vi "Replace String in File.vi"(7 "File Path":path, 8 "error in":errorcluster, 9 "Replace String":string, 10 "Search String":string, 11 "IFile Manager in":refnum<class "Mock IFile Manager.lvclass">) -> (0 "error out":errorcluster, 3 "IFile Manager out":refnum<class "Mock IFile Manager.lvclass">)   [LabVIEW 2026, in "Mock IFile Manager.lvclass"]
doc: "This VI replaces all instances of the search string by the replace strin in the provided text file."
uses:
  Mock IFile Manager.lvclass
  C:/Program Files/National Instruments/LabVIEW 2026/vi.lib/Astemes/LMock/Mock.lvclass
  Mock IFile Manager.lvclass/Mock IFile Manager.ctl
  <vilib>/Astemes/LMock/Mock.lvclass
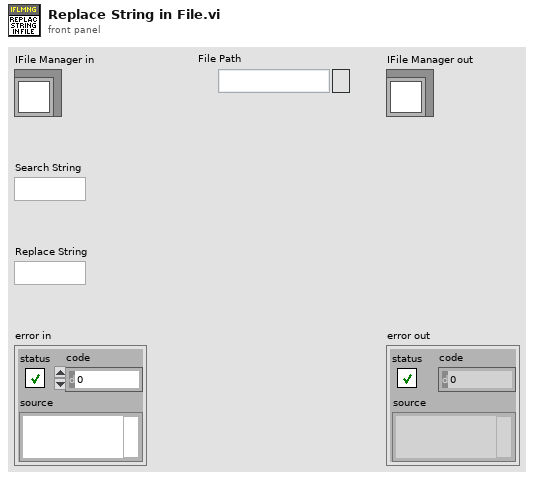
[diagram p1: front panel]
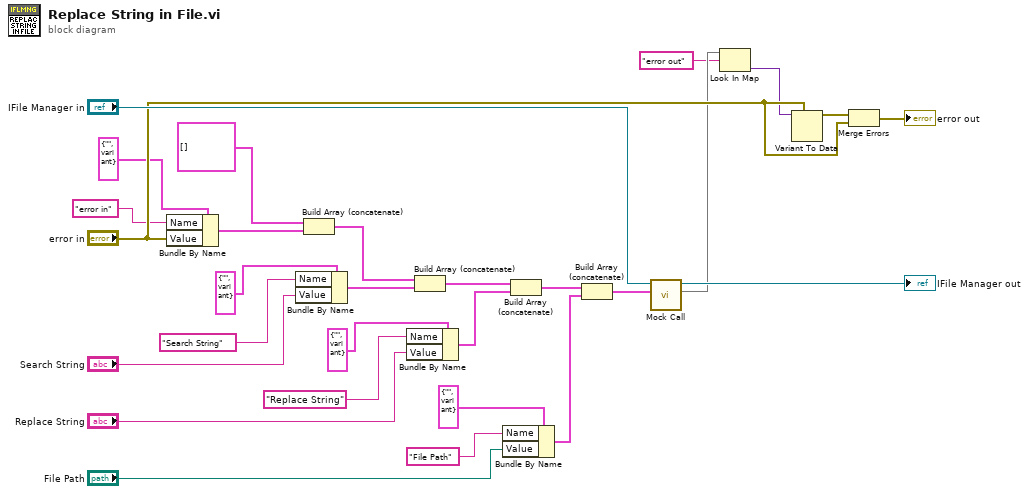
[diagram p0: block diagram]
diagram:
  n1 = Bundle By Name(cluster=cluster{"Name":string, "Value":variant} {"Name"="", "Value"=variant} ("element"), "Name"="error in", "Value"="error in") -> (w7:cluster{"Name":string, "Value":variant})
  n2 = Bundle By Name(cluster=cluster{"Name":string, "Value":variant} {"Name"="", "Value"=variant} ("element"), "Name"="Search String", "Value"="Search String") -> (w5:cluster{"Name":string, "Value":variant})
  n3 = Build Array (concatenate)(cluster{"Name":string, "Value":variant}[] [] ("Control Values"), w7) -> (w16:cluster{"Name":string, "Value":variant}[])
  n4 = Bundle By Name(cluster=cluster{"Name":string, "Value":variant} {"Name"="", "Value"=variant} ("element"), "Name"="Replace String", "Value"="Replace String") -> (w3:cluster{"Name":string, "Value":variant})
  n5 = Build Array (concatenate)(w16, w5) -> (w19:cluster{"Name":string, "Value":variant}[])
  n6 = Bundle By Name(cluster=cluster{"Name":string, "Value":variant} {"Name"="", "Value"=variant} ("element"), "Name"="File Path", "Value"="File Path") -> (w1:cluster{"Name":string, "Value":variant})
  n7 = Build Array (concatenate)(w19, w3) -> (w22:cluster{"Name":string, "Value":variant}[])
  n8 = Build Array (concatenate)(w22, w1) -> (w25:cluster{"Name":string, "Value":variant}[])
  n9 = call <vilib>:"Mock Call.vi"("Control Values"=w25, "Mock In"="IFile Manager in") -> ("Return Values"=w14:map{string, variant}, "Mock Out"=→"IFile Manager out":refnum<class "Mock IFile Manager.lvclass">)  [unwired: 8 in]
  n10 = Look In Map(map=w14, key="error out") -> (value=w12:variant)  [unwired: 1 in, 1 out]
  n11 = Variant To Data(type="error in", Variant=w12) -> (data=w11:errorcluster)  [unwired: 1 in, 1 out]
  n12 = Merge Errors(w11, "error in") -> (→"error out":errorcluster)
